vi "Enqueue Frame.vi"(8 "error in":errorcluster, 10 "GUID":string, 11 "Data":string[][](array[string])) -> (0 "error out":errorcluster, 3 "overflow?":bool)   [LabVIEW 2025, in "CAN-LIN Raw Bus Capture.lvclass"]
uses:
  CAN-LIN Raw Bus Capture.lvclass
  CAN-LIN Raw Bus Capture.lvclass/CAN-LIN Raw Bus Capture.ctl
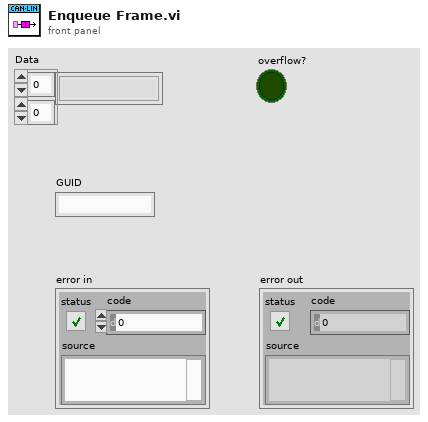
[diagram p1: front panel]
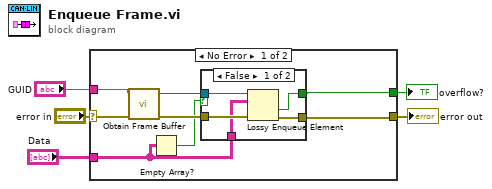
[diagram p0: block diagram]
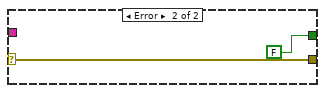
[diagram p3: hidden frame]
diagram:
  n1 = case shown="No Error" "error in" {
    selector: "error in" -> [w13 w21]
    tunnel: [w11 w21] -> w4
    tunnel: "Data" -> [w8 _]
    tunnel: [w9 FALSE ("overflow?")] -> w2
    tunnel: "GUID" -> [w6 _]
    frame No Error {
      n2 = call "Obtain Frame Buffer.vi"("error in"=w13, "GUID"=w6) -> ("error out"=w12:errorcluster, "queue out"=w10:refnum<queue>)  [unwired: 8 in]
      n3 = Empty Array?(array=w8) -> (empty?=w7:bool)
      n4 = case shown="False" w7 {
        tunnel: w12 -> [w18 w19]
        tunnel: [w17 w19] -> w11
        tunnel: w10 -> [w16 _]
        tunnel: w8 -> [w15 _]
        tunnel: [w14 _] -> w9
        frame False {
          n5 = Lossy Enqueue Element(queue=w16, element=w15, error in (no error)=w18) -> (overflow?=w14:bool, error out=w17:errorcluster)  [unwired: 2 out]
        }
        frame True {
        }
      }
    }
    frame Error {
    }
  }
  "error out" <- w4
  "overflow?" <- w2
